vi "Sim First Order Step.vi"(9 "dt s":dbl=0.1, 10 "Setpoints":T1[](array[typedef]), 11 "State":T1[](array[typedef])) -> (3 "new State":T1[](array[typedef]))   [LabVIEW 2026]
doc: "One integration step of the simulated rig: every State channel moves toward its setpoint as a first-order lag, tau by channel name (Pressure 0.8, Flow 0.6, Displacement 0.3, other 0.5). A State channel with no setpoint keeps its value; every setpoint channel not present in State is appended, starting from 0 and integrated once. Pure function, no error terminals, AF-free."
uses:
  src/Typedefs/Channel Value.ctl
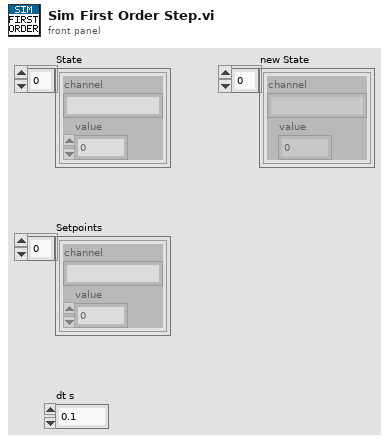
[diagram p1: front panel]
types:
  T1 = typedef "Channel Value.ctl" = cluster{"channel":string, "value":dbl}
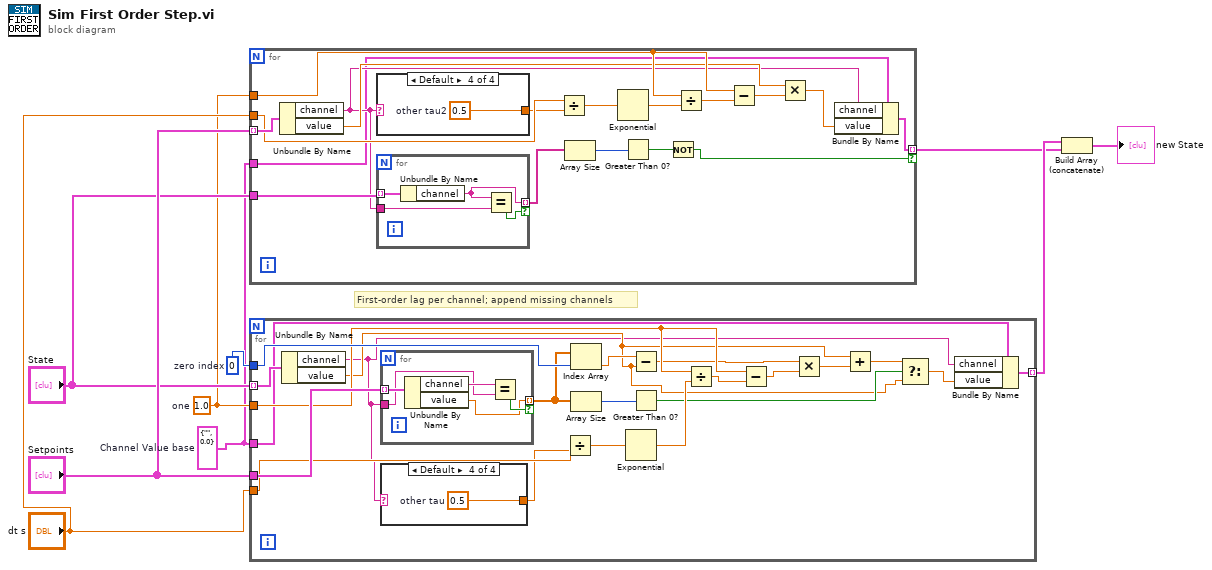
[diagram p0: block diagram]
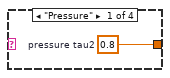
[diagram p2: hidden frame]
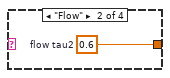
[diagram p3: hidden frame]
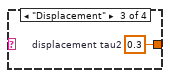
[diagram p4: hidden frame]
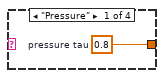
[diagram p5: hidden frame]
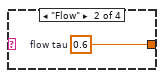
[diagram p6: hidden frame]
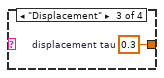
[diagram p7: hidden frame]
diagram:
  w4 = cluster{"channel":string, "value":dbl} {"channel"="", "value"=0.0}  # Channel Value base
  w9 = 0  # zero index
  w5 = 1.0  # one
  # "First-order lag per channel; append missing channels"
  n1 = for {
    tunnel: "Setpoints" -> [w27] mode=indexing
    tunnel: "State" -> [w26]
    tunnel: "dt s" -> [w22]
    tunnel: w5 -> [w18]
    tunnel: w4 -> [w12]
    tunnel: [w10] -> w2 mode=indexing if=w11
    n2 = Unbundle By Name(w27) -> ("channel"=w14:string, "value"=w16:dbl)
    n3 = case shown="Default" w14 {
      tunnel: [w28 w29 w30 w31] -> w21
      frame "Pressure" {
        w28 = 0.8  # pressure tau2
      }
      frame "Flow" {
        w29 = 0.6  # flow tau2
      }
      frame "Displacement" {
        w30 = 0.3  # displacement tau2
      }
      frame Default {
        w31 = 0.5  # other tau2
      }
    }
    n4 = for {
      tunnel: w26 -> [w35] mode=indexing
      tunnel: w14 -> [w34]
      tunnel: [w32] -> w25 mode=indexing if=w33
      n5 = Unbundle By Name(w35) -> ("channel"=w32:string)
      n6 = Equal?(x=w32, y=w34) -> (x = y?=w33:bool)
    }
    n7 = Divide(x=w22, y=w21) -> (x/y=w20:dbl)
    n8 = Array Size(array=w25) -> (size(s)=w24:i32)
    n9 = Exponential(1:w20) -> (0:w19:dbl)
    n10 = Greater Than 0?(x=w24) -> (x > 0?=w23:bool)
    n11 = Not(x=w23) -> (.not. x?=w11:bool)
    n12 = Divide(x=w18, y=w19) -> (x/y=w17:dbl)
    n13 = Subtract(x=w18, y=w17) -> (x-y=w15:dbl)
    n14 = Multiply(x=w16, y=w15) -> (x*y=w13:dbl)
    n15 = Bundle By Name(cluster=w12, "channel"=w14, "value"=w13) -> (w10:cluster{"channel":string, "value":dbl})
  }
  n16 = for {
    tunnel: "State" -> [w57] mode=indexing
    tunnel: "Setpoints" -> [w56]
    tunnel: "dt s" -> [w52]
    tunnel: w5 -> [w48]
    tunnel: w9 -> [w55]
    tunnel: w4 -> [w37]
    tunnel: [w36] -> w3 mode=indexing
    n17 = Unbundle By Name(w57) -> ("channel"=w39:string, "value"=w40:dbl)
    n18 = for {
      tunnel: w56 -> [w66] mode=indexing
      tunnel: w39 -> [w64]
      tunnel: [w62] -> w54 mode=indexing if=w63
      n19 = Unbundle By Name(w66) -> ("channel"=w65:string, "value"=w62:dbl)
      n20 = Equal?(x=w65, y=w64) -> (x = y?=w63:bool)
    }
    n21 = case shown="Default" w39 {
      tunnel: [w58 w59 w60 w61] -> w51
      frame "Pressure" {
        w58 = 0.8  # pressure tau
      }
      frame "Flow" {
        w59 = 0.6  # flow tau
      }
      frame "Displacement" {
        w60 = 0.3  # displacement tau
      }
      frame Default {
        w61 = 0.5  # other tau
      }
    }
    n22 = Divide(x=w52, y=w51) -> (x/y=w50:dbl)
    n23 = Index Array(array=w54, index=w55) -> (element=w46:dbl)
    n24 = Array Size(array=w54) -> (size(s)=w53:i32)
    n25 = Exponential(1:w50) -> (0:w49:dbl)
    n26 = Subtract(x=w46, y=w40) -> (x-y=w45:dbl)
    n27 = Greater Than 0?(x=w53) -> (x > 0?=w41:bool)
    n28 = Divide(x=w48, y=w49) -> (x/y=w47:dbl)
    n29 = Subtract(x=w48, y=w47) -> (x-y=w44:dbl)
    n30 = Multiply(x=w45, y=w44) -> (x*y=w43:dbl)
    n31 = Add(x=w40, y=w43) -> (x+y=w42:dbl)
    n32 = Select(t=w42, s=w41, f=w40) -> (s? t:f=w38:dbl)
    n33 = Bundle By Name(cluster=w37, "channel"=w39, "value"=w38) -> (w36:cluster{"channel":string, "value":dbl})
  }
  n34 = Build Array (concatenate)(w3, w2) -> (→"new State":cluster{"channel":string, "value":dbl}[])
